vi "Set NodeIDs.vi"(8 "error in (no error)":errorcluster, 10 "PLC Folder Names":string[](array[string]), 11 "AbstractUUT":refnum<class "Abstract.lvclass">=refnum) -> (0 "error out":errorcluster, 3 "AbstractUUT out":refnum<class "Abstract.lvclass">)   [LabVIEW 2025, in "Abstract.lvclass"]
uses:
  Abstract.lvclass
  Abstract.lvclass/Abstract.ctl
  Read OPC UA Ref.vi
  Read Subscription.vi
  Write NodeIDs.vi
  Read Rx from PLC.vi
  Read Tx to PLC.vi
  <vilib>/OPCUA/NI OPC UA Client.lvlib
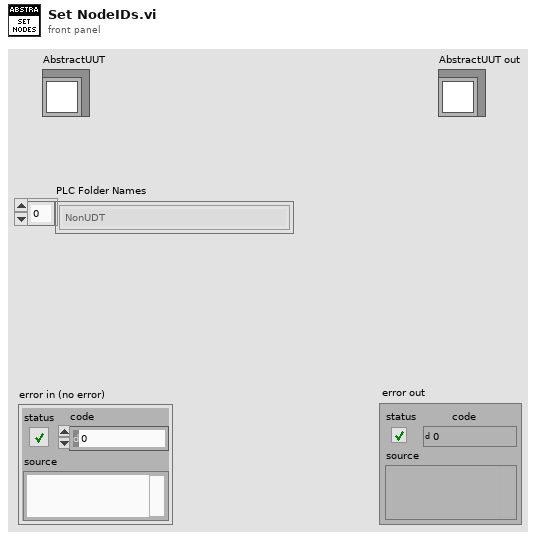
[diagram p1: front panel]
types:
  T1 = typedef "OPC UA Client Refnum.ctl" = refnum<k21>
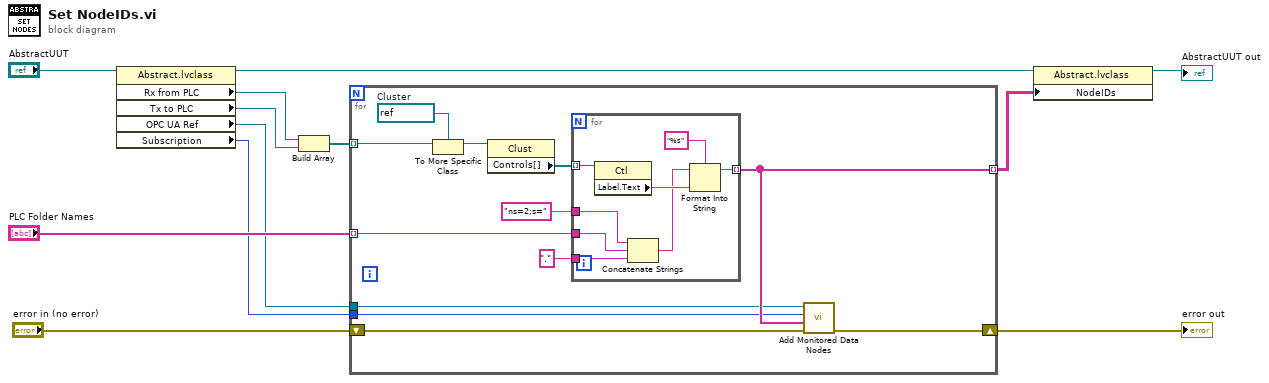
[diagram p0: block diagram]
diagram:
  n1 = property class="Abstract.lvclass"(reference="AbstractUUT") -> (reference out=w7:refnum<class "Abstract.lvclass">, "Rx from PLC"=w4:refnum<vi>, "Tx to PLC"=w6:refnum<vi>, "OPC UA Ref"=w3:T1, "Subscription"=w2:u32)  [unwired: 1 in, 1 out]
  n2 = Build Array(w4, w6) -> (w10:refnum<vi>[])
  n3 = for {
    tunnel: [w15] -> w8 mode=indexing
    tunnel: "PLC Folder Names" -> [w24] mode=indexing
    tunnel: w10 -> [w21] mode=indexing
    shift-right: [w16] -> w1
    shift-left: "error in (no error)" -> [w17]
    tunnel: w3 -> [w14]
    tunnel: w2 -> [w13]
    w18 = refnum<vi> refnum  # Cluster
    n4 = To More Specific Class(target class=w18, reference=w21) -> (specific class reference=w22:refnum<vi>)  [unwired: 1 in, 1 out]
    n5 = property class="Clust"(reference=w22) -> ("Controls[]"=w23:refnum<vi>[])  [unwired: 1 in, 2 out]
    n6 = for {
      tunnel: w23 -> [w32] mode=indexing
      tunnel: w24 -> [w28]
      tunnel: [w29] -> w15 mode=indexing
      tunnel: "ns=2;s=" ("format string") -> [w27]
      tunnel: "." ("Deliminated Char") -> [w25]
      n7 = property class="Ctl"(reference=w32) -> ("Label.Text"=w31:string)  [unwired: 1 in, 2 out]
      n8 = Concatenate Strings(w27, w28, w25) -> (w26:string)
      n9 = Format Into String(format string="%s", initial string=w26, w31) -> (resulting string=w29:string)  [unwired: 1 in, 1 out]
    }
    n10 = call <vilib>:"Add Monitored Data Nodes.vi"("error in (no error)"=w17, "node IDs"=w15, "subscription ID in"=w13, "OPC UA client refnum in"=w14) -> ("error out"=w16:errorcluster)  [unwired: 4 in, 3 out]
  }
  "error out" <- w1
  n11 = property class="Abstract.lvclass"(reference=w7, "NodeIDs"=w8) -> (reference out=→"AbstractUUT out":refnum<class "Abstract.lvclass">)  [unwired: 1 in, 1 out]
